vi "Create Low Pass Filter (FGV).vi"(6 "fs (Hz)":dbl, 7 "init [F]":bool, 8 "error in (no error)":errorcluster, 9 "Low Pass Cutoff (Hz)":dbl, 11 "order":i32=2) -> (0 "error out":errorcluster, 3 "IIR Filters":T1(array[cluster]), 5 "init out":bool)   [LabVIEW 2019, in "DSP.lvclass"]
uses:
  DSP.lvclass
  <vilib>/Analysis/3filter.llb/Filter Passband Type.ctl
  <vilib>/Analysis/NI_AALBase.lvlib
panel:
  out "concatenated string":string
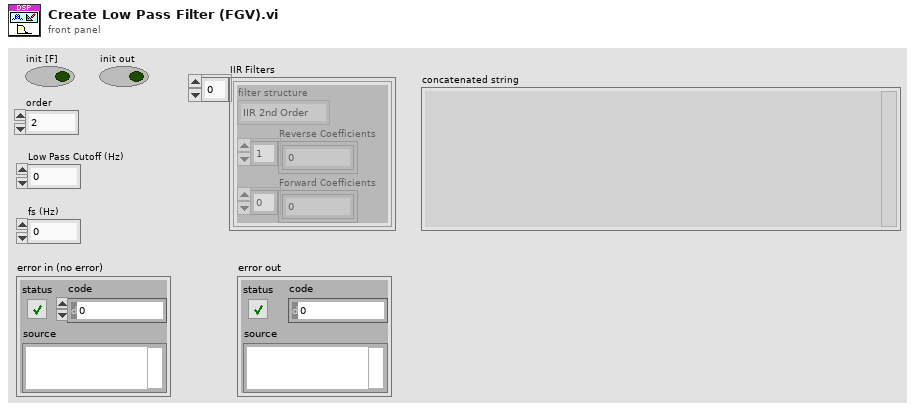
[diagram p1: front panel]
types:
  T1 = cluster{"filter structure":enum32{"IIR 2nd Order", "IIR 4th Order"}, "Reverse Coefficients":dbl[], "Forward Coefficients":dbl[]}[]
  T2 = typedef "NI_AALBase.lvlib/Filter Passband Type.ctl" = enum32{"Lowpass", "Highpass", "Bandpass", "Bandstop"}
  T3 = cluster{"filter structure":enum32{"IIR 2nd Order", "IIR 4th Order"}, "Reverse Coefficients":dbl[], "Forward Coefficients":dbl[]}
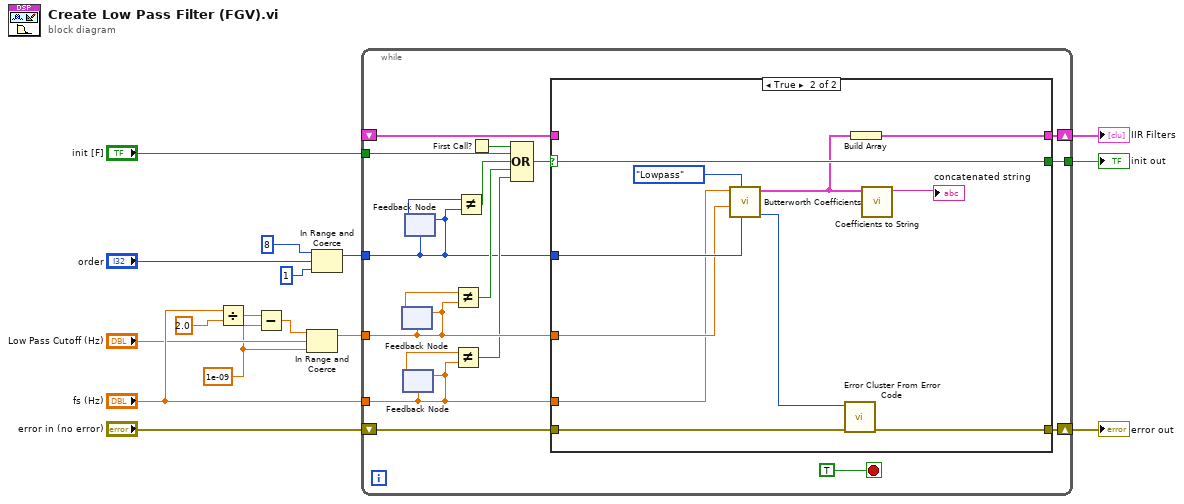
[diagram p0: block diagram]
diagram:
  w2 = 1e-09 ("lower limit")
  n1 = Divide(x="fs (Hz)", y=2.0 ("lower limit")) -> (x/y=w14:dbl)
  n2 = Subtract(x=w14, y=w2) -> (x-y=w13:dbl)
  n3 = In Range and Coerce(upper limit=w13, x="Low Pass Cutoff (Hz)", lower limit=w2) -> (coerced(x)=w9:dbl)  [unwired: 1 out]
  n4 = In Range and Coerce(upper limit=8, x="order", lower limit=1) -> (coerced(x)=w5:i32)  [unwired: 1 out]
  n5 = while {
    tunnel: w9 -> [w23]
    tunnel: "fs (Hz)" -> [w26]
    shift-right: [w32] -> w16
    shift-left: "error in (no error)" -> [w33]
    shift-right: [w34] -> w1
    shift-left: _ -> [w29]
    tunnel: "init [F]" -> [w28]
    tunnel: w5 -> [w19]
    tunnel: [w17] -> w3
    stop <- TRUE stop-if-true
    n6 = feedback #1(w23) -> (w24:dbl)
    n7 = feedback-in #1(w23) -> ()
    n8 = feedback #2(w26) -> (w25:dbl)
    n9 = feedback-in #2(w26) -> ()
    n10 = feedback #3(w19) -> (w22:i32)
    n11 = feedback-in #3(w19) -> ()
    n12 = Not Equal?(x=w24, y=w23) -> (x != y?=w30:bool)
    n13 = Not Equal?(x=w25, y=w26) -> (x != y?=w21:bool)
    n14 = Not Equal?(x=w22, y=w19) -> (x != y?=w20:bool)
    n15 = First Call?() -> (First Call?: T/F=w18:bool)
    n16 = Compound Arithmetic op=OR(w18, w28, w20, w30, w21) -> (w27:bool)
    n17 = case shown="True" w27 {
      selector: w27 -> [w35 w48]
      tunnel: [w37 w43] -> w34
      tunnel: w33 -> [w36 w45]
      tunnel: [w36 w46] -> w32
      tunnel: w23 -> [_ w41]
      tunnel: w26 -> [_ w39]
      tunnel: w29 -> [w37 _]
      tunnel: w19 -> [_ w42]
      tunnel: [w35 w48] -> w17
      frame False {
      }
      frame True {
        n18 = call <vilib>:"Butterworth Coefficients.vi"("order"=w42, "filter type"=Filter_Passband_Type."Lowpass", "low cutoff freq: fl"=w41, "sampling freq: fs"=w39) -> ("error"=w44:i32, "IIR Filter Cluster"=w38:T3)  [unwired: 6 in]
        n19 = call <vilib>:"Error Cluster From Error Code.vi"("error in (no error)"=w45, "error code (0)"=w44) -> ("error out"=w46:errorcluster)  [unwired: 7 in]
        n20 = Build Array(w38) -> (w43:T1)
        n21 = call "Coefficients to String.vi"("IIR Filter Cluster"=w38) -> ("String"=→"concatenated string":string)  [unwired: 10 in]
      }
    }
  }
  "init out" <- w3
  "IIR Filters" <- w1
  "error out" <- w16
